vi "PathPlanner_Path_Equals.vi"(9 "Other Path":T1={"Reversed"=FALSE, "RotationTargets"=[], "ConstraintZones"=[], "EventMarkers"=[], "GlobalConstraints"={"MaxVelocityMps;"=0.0, "MaxAccelerationMpsSq;"=0.0, "MaxAngularVelRadPsEc;"=0.0, "MaxAngularAccRadPSecSq"=0.0, "Exists"=FALSE, "Unlimited"=FALSE, "NominalVoltageVolts"=12.0}, "GoalEndState"={"VelocityMPS"=0.0, "Rotation"={"VALUE"=0.0, "COS"=1.0, "SIN"=0.0}}, "AllPoints"=[], "Name"="", "Waypoints"=[], "PointTowardsZones"=[], "IdealStartingState"={"VelocityMPS"=0.0, "Rotation"={"VALUE"=1.0, "COS"=0.0, "SIN"=0.0}}, "IsChoreoPath"=FALSE, "PreventFlipping"=FALSE} {"IdealStartingState"."Rotation"."SIN" format="%13.4f"; "IdealStartingState"."Rotation"."COS" format="%13.4f"; "IdealStartingState"."Rotation"."VALUE" format="%13.4f"; "PointTowardsZones"."TargetPosition"."Y" format="%14.3f"; "PointTowardsZones"."TargetPosition"."X" format="%14.3f"; "PointTowardsZones"."RotationOffset"."SIN" format="%13.4f"; "PointTowardsZones"."RotationOffset"."COS" format="%13.4f"; "PointTowardsZones"."RotationOffset"."VALUE" format="%13.4f"; "Waypoints"."nextControl"."Y" format="%14.3f"; "Waypoints"."nextControl"."X" format="%14.3f"; "Waypoints"."anchor"."Y" format="%14.3f"; "Waypoints"."anchor"."X" format="%14.3f"; "Waypoints"."prevControl"."Y" format="%14.3f"; "Waypoints"."prevControl"."X" format="%14.3f"; "AllPoints"."RotationTarget"."rotation"."SIN" format="%13.4f"; "AllPoints"."RotationTarget"."rotation"."COS" format="%13.4f"; "AllPoints"."RotationTarget"."rotation"."VALUE" format="%13.4f"; "AllPoints"."Position"."Y" format="%14.3f"; "AllPoints"."Position"."X" format="%14.3f"; "GoalEndState"."Rotation"."SIN" format="%13.4f"; "GoalEndState"."Rotation"."COS" format="%13.4f"; "GoalEndState"."Rotation"."VALUE" format="%13.4f"; "RotationTargets"."rotation"."SIN" format="%13.4f"; "RotationTargets"."rotation"."COS" format="%13.4f"; "RotationTargets"."rotation"."VALUE" format="%13.4f"}, 11 "Path":T1={"Reversed"=FALSE, "RotationTargets"=[], "ConstraintZones"=[], "EventMarkers"=[], "GlobalConstraints"={"MaxVelocityMps;"=0.0, "MaxAccelerationMpsSq;"=0.0, "MaxAngularVelRadPsEc;"=0.0, "MaxAngularAccRadPSecSq"=0.0, "Exists"=FALSE, "Unlimited"=FALSE, "NominalVoltageVolts"=12.0}, "GoalEndState"={"VelocityMPS"=0.0, "Rotation"={"VALUE"=0.0, "COS"=1.0, "SIN"=0.0}}, "AllPoints"=[], "Name"="", "Waypoints"=[], "PointTowardsZones"=[], "IdealStartingState"={"VelocityMPS"=0.0, "Rotation"={"VALUE"=1.0, "COS"=0.0, "SIN"=0.0}}, "IsChoreoPath"=FALSE, "PreventFlipping"=FALSE} {"IdealStartingState"."Rotation"."SIN" format="%13.4f"; "IdealStartingState"."Rotation"."COS" format="%13.4f"; "IdealStartingState"."Rotation"."VALUE" format="%13.4f"; "PointTowardsZones"."TargetPosition"."Y" format="%14.3f"; "PointTowardsZones"."TargetPosition"."X" format="%14.3f"; "PointTowardsZones"."RotationOffset"."SIN" format="%13.4f"; "PointTowardsZones"."RotationOffset"."COS" format="%13.4f"; "PointTowardsZones"."RotationOffset"."VALUE" format="%13.4f"; "Waypoints"."nextControl"."Y" format="%14.3f"; "Waypoints"."nextControl"."X" format="%14.3f"; "Waypoints"."anchor"."Y" format="%14.3f"; "Waypoints"."anchor"."X" format="%14.3f"; "Waypoints"."prevControl"."Y" format="%14.3f"; "Waypoints"."prevControl"."X" format="%14.3f"; "AllPoints"."RotationTarget"."rotation"."SIN" format="%13.4f"; "AllPoints"."RotationTarget"."rotation"."COS" format="%13.4f"; "AllPoints"."RotationTarget"."rotation"."VALUE" format="%13.4f"; "AllPoints"."Position"."Y" format="%14.3f"; "AllPoints"."Position"."X" format="%14.3f"; "GoalEndState"."Rotation"."SIN" format="%13.4f"; "GoalEndState"."Rotation"."COS" format="%13.4f"; "GoalEndState"."Rotation"."VALUE" format="%13.4f"; "RotationTargets"."rotation"."SIN" format="%13.4f"; "RotationTargets"."rotation"."COS" format="%13.4f"; "RotationTargets"."rotation"."VALUE" format="%13.4f"}) -> (3 "Equals":bool)   [LabVIEW 2019, in "PathPlanner24.lvlib"]
doc: "Determines if two paths are identical.\n\nNote: Reversed and PreviewEndState are not part of the comparison\n\nInputs:\n - Path Path - Data structure containing path definition\n - OtherPath - Path - Data structure containing path definition\n\nOutputs:\n - Equal - boolean - TRUE if paths are identical."
uses:
  PathPlanner24.lvlib
  <vilib>/Rock Robotics/WPI/ThirdParty/JAS_Junk/TrajLib/TypeDef/TRANSLATION2D.ctl
  <vilib>/Rock Robotics/WPI/ThirdParty/JAS_Junk/TrajLib/Trajectory_Library.lvlib
  <vilib>/Rock Robotics/WPI/ThirdParty/JAS_Junk/TrajLib/TypeDef/ROTATION2D.ctl
  TypeDef/PathPlannerRotationTarget.ctl
  TypeDef/PathPlannerPathConstraints.ctl
  TypeDef/PathPlannerConstraintsZone.ctl
  TypeDef/PathPlannerCommandUtil.ctl
  TypeDef/PathPlannerEventMarker.ctl
  TypeDef/PathPlannerGoalEndState.ctl
  TypeDef/PathPlannerPathPoint.ctl
  TypeDef/PathPlannerPath.ctl
  ENum/PathPlanner_TrajectoryEvent_Type_ENUM.ctl
  TypeDef/PathPlannerWaypoint.ctl
  TypeDef/PathPlannerPointTowardsZone.ctl
  TypeDef/PathPlannerIdealStartingState.ctl
  ENum/PathPlanner_CommandUtil_Type_ENUM.ctl
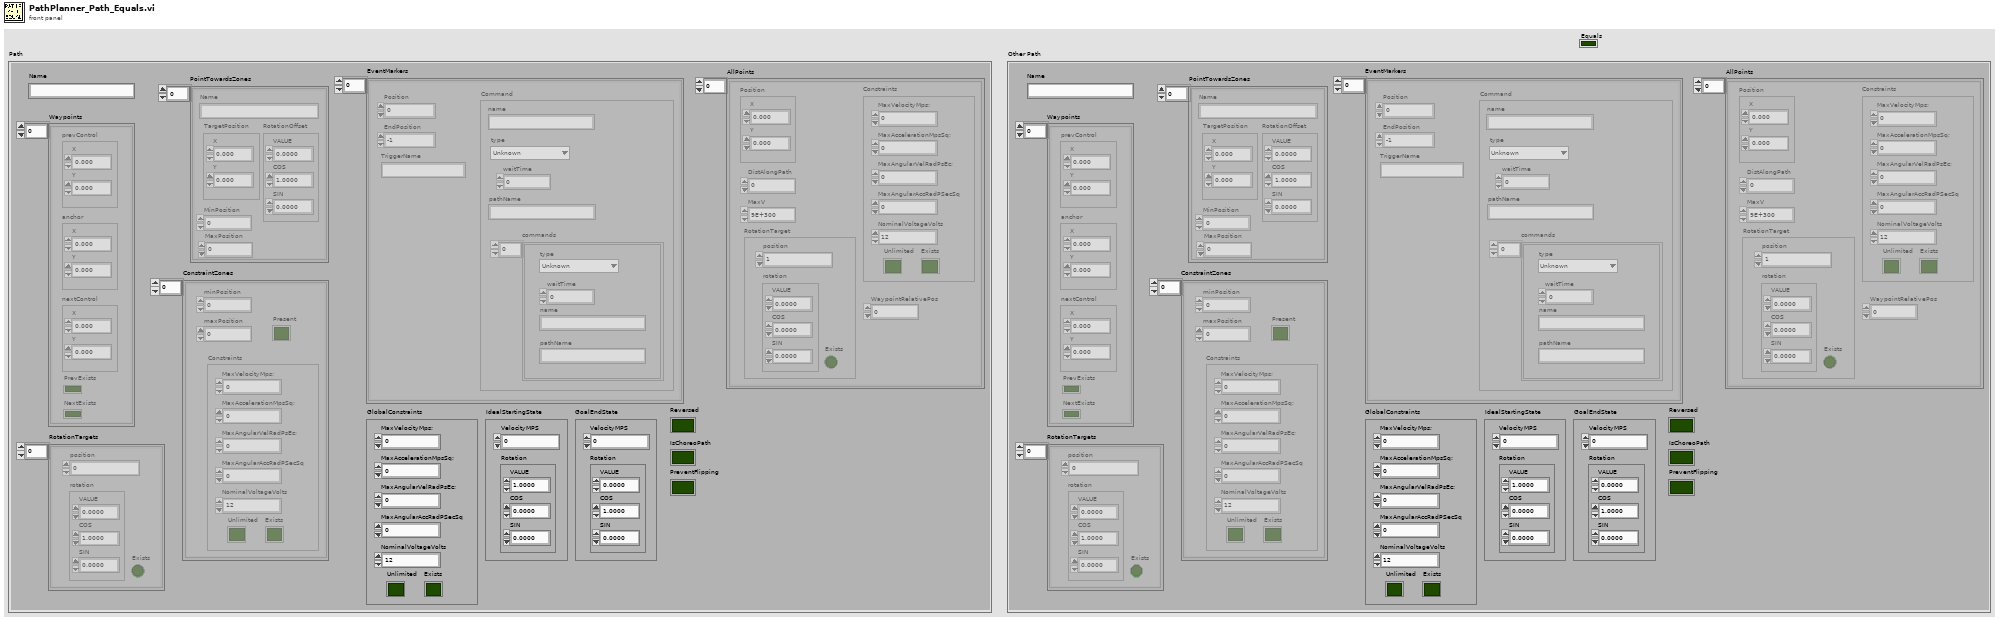
[diagram p1: front panel]
types:
  T1 = typedef "PathPlanner24.lvlib/PathPlannerPath.ctl" = cluster{"Reversed":bool, "RotationTargets":T2[], "ConstraintZones":T4[], "EventMarkers":T6[], "GlobalConstraints":T5, "GoalEndState":T10, "AllPoints":T11[], "Name":string, "Waypoints":T13[], "PointTowardsZones":T14[], "IdealStartingState":T15, "IsChoreoPath":bool, "PreventFlipping":bool}
  T2 = typedef "PathPlanner24.lvlib/PathPlannerRotationTarget.ctl" = cluster{"position":dbl, "rotation":T3, "Exists":bool}
  T3 = typedef "Trajectory_Library.lvlib/ROTATION2D.ctl" = cluster{"VALUE":dbl, "COS":dbl, "SIN":dbl}
  T4 = typedef "PathPlanner24.lvlib/PathPlannerConstraintsZone.ctl" = cluster{"minPosition":dbl, "maxPosition":dbl, "Constraints":T5, "Present":bool}
  T5 = typedef "PathPlanner24.lvlib/PathPlannerPathConstraints.ctl" = cluster{"MaxVelocityMps;":dbl, "MaxAccelerationMpsSq;":dbl, "MaxAngularVelRadPsEc;":dbl, "MaxAngularAccRadPSecSq":dbl, "Exists":bool, "Unlimited":bool, "NominalVoltageVolts":dbl}
  T6 = typedef "PathPlanner24.lvlib/PathPlannerEventMarker.ctl" = cluster{"Position":dbl, "Command":T7, "TriggerName":string, "EndPosition":dbl}
  T7 = typedef "PathPlanner24.lvlib/PathPlannerCommandUtil.ctl" = cluster{"waitTime":dbl, "name":string, "pathName":string, "commands":cluster{"type":T8, "waitTime":dbl, "name":string, "pathName":string}[], "type":T9}
  T8 = typedef "PathPlanner24.lvlib/PathPlanner_TrajectoryEvent_Type_ENUM.ctl" = enum16{"Unknown", "Wait", "Named", "Path", "Sequential", "Parallel", "Race", "Deadline", "PointTowardsZoneEnter", "PointTowardsZoneExit", "TriggerEventStart", "TriggerEventStop", "TriggerEventOneshot"}
  T9 = typedef "PathPlanner24.lvlib/PathPlanner_CommandUtil_Type_ENUM.ctl" = enum16{"Unknown", "Wait", "Named", "Path", "Sequential", "Parallel", "Race", "Deadline"}
  T10 = typedef "PathPlanner24.lvlib/PathPlannerGoalEndState.ctl" = cluster{"VelocityMPS":dbl, "Rotation":T3}
  T11 = typedef "PathPlanner24.lvlib/PathPlannerPathPoint.ctl" = cluster{"Position":T12, "DistAlongPath":dbl, "MaxV":dbl, "Constraints":T5, "RotationTarget":T2, "WaypointRelativePos":dbl}
  T12 = typedef "Trajectory_Library.lvlib/TRANSLATION2D.ctl" = cluster{"X":dbl, "Y":dbl}
  T13 = typedef "PathPlanner24.lvlib/PathPlannerWaypoint.ctl" = cluster{"prevControl":T12, "anchor":T12, "nextControl":T12, "PrevExists":bool, "NextExists":bool}
  T14 = typedef "PathPlanner24.lvlib/PathPlannerPointTowardsZone.ctl" = cluster{"RotationOffset":T3, "Name":string, "TargetPosition":T12, "MinPosition":dbl, "MaxPosition":dbl}
  T15 = typedef "PathPlanner24.lvlib/PathPlannerIdealStartingState.ctl" = cluster{"VelocityMPS":dbl, "Rotation":T3}
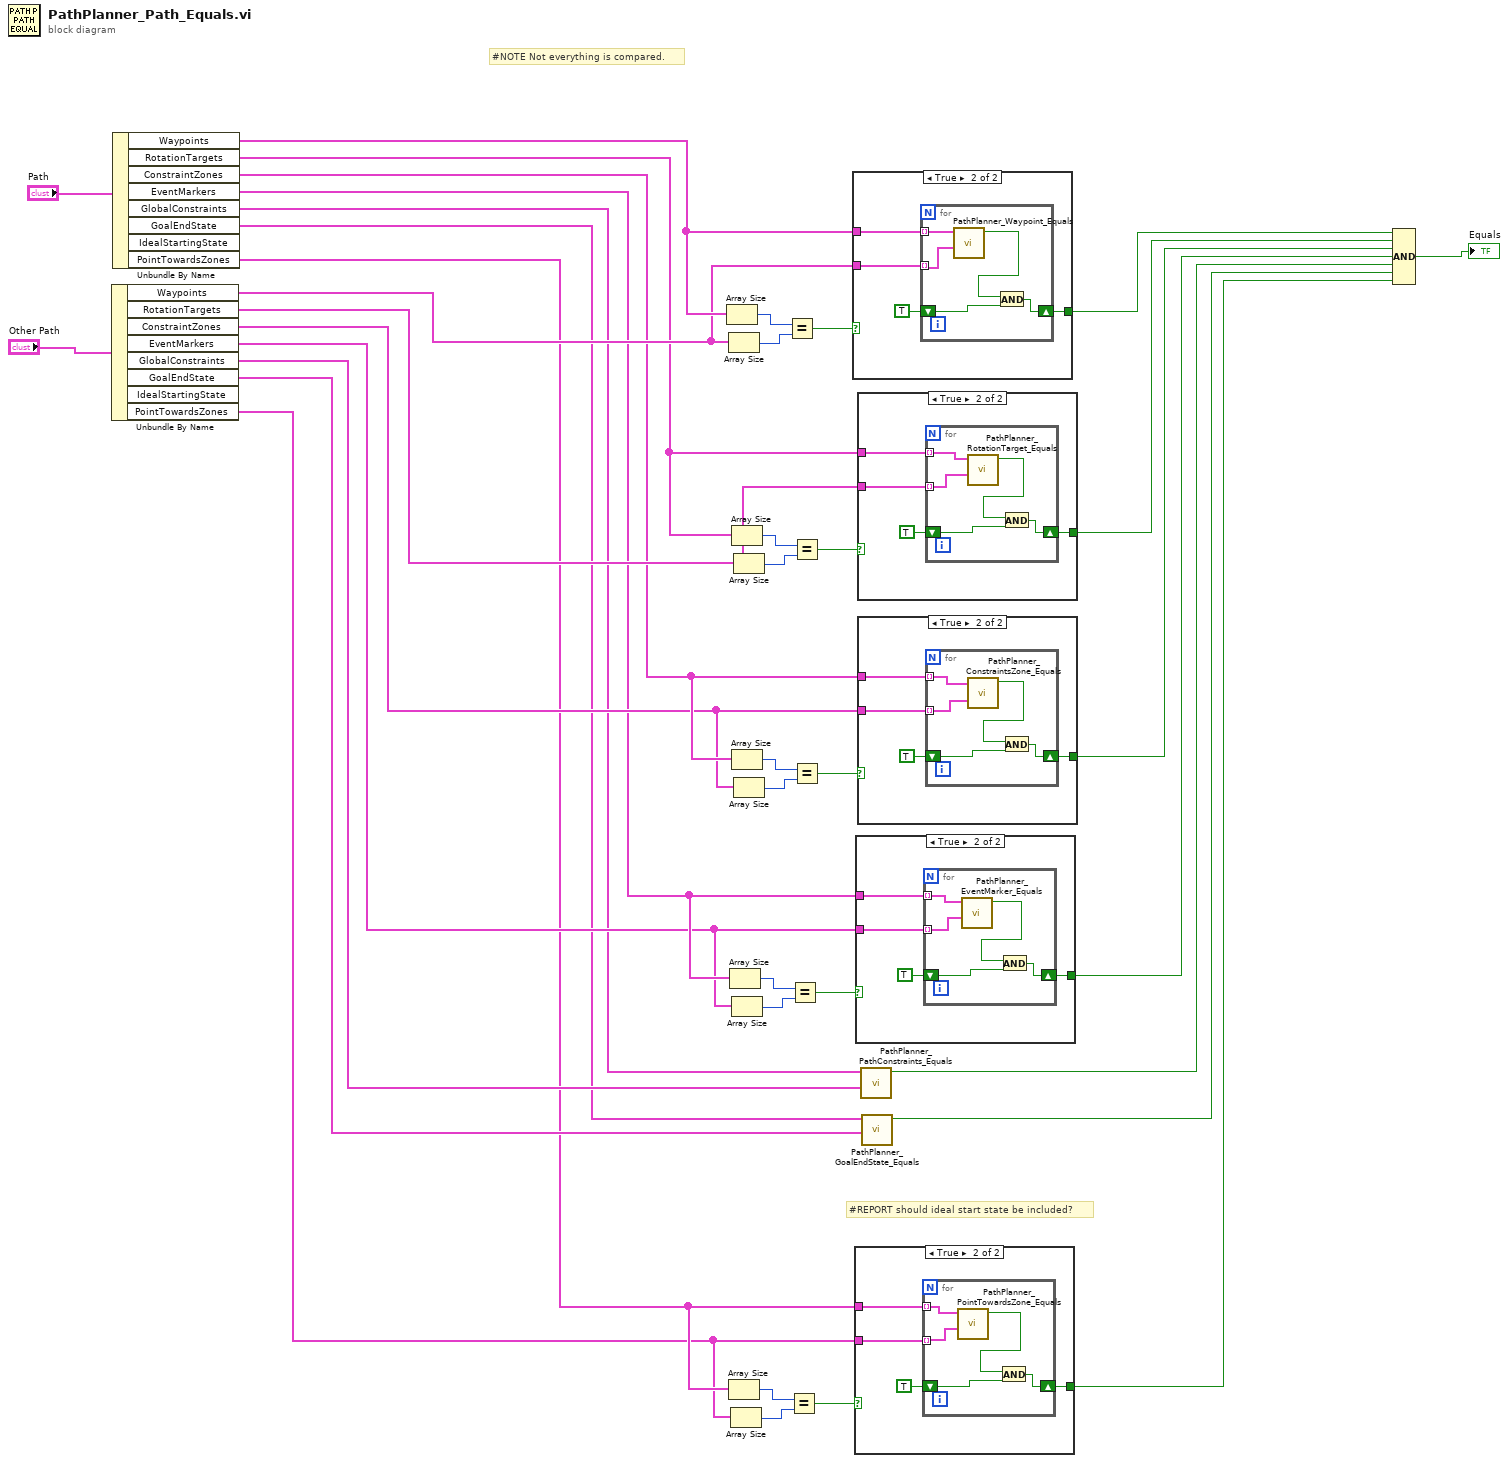
[diagram p0: block diagram]
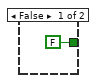
[diagram p2: hidden frame]
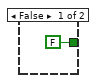
[diagram p3: hidden frame]
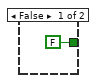
[diagram p4: hidden frame]
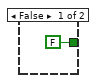
[diagram p5: hidden frame]
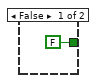
[diagram p6: hidden frame]
diagram:
  # "#REPORT should ideal start state be included?"
  # "#NOTE Not everything is compared."
  n1 = Unbundle By Name("Other Path") -> ("Waypoints"=w33:T13[], "RotationTargets"=w26:T2[], "ConstraintZones"=w20:T4[], "EventMarkers"=w14:T6[], "GlobalConstraints"=w11:T5, "GoalEndState"=w8:T10, "PointTowardsZones"=w2:T14[])  [unwired: 1 out]
  n2 = Unbundle By Name("Path") -> ("Waypoints"=w34:T13[], "RotationTargets"=w27:T2[], "ConstraintZones"=w21:T4[], "EventMarkers"=w15:T6[], "GlobalConstraints"=w12:T5, "GoalEndState"=w9:T10, "PointTowardsZones"=w3:T14[])  [unwired: 1 out]
  n3 = Array Size(array=w34) -> (size(s)=w37:i32)
  n4 = Array Size(array=w33) -> (size(s)=w36:i32)
  n5 = Array Size(array=w3) -> (size(s)=w6:i32)
  n6 = Array Size(array=w15) -> (size(s)=w18:i32)
  n7 = Array Size(array=w2) -> (size(s)=w5:i32)
  n8 = Array Size(array=w27) -> (size(s)=w30:i32)
  n9 = Array Size(array=w21) -> (size(s)=w24:i32)
  n10 = Array Size(array=w14) -> (size(s)=w17:i32)
  n11 = Array Size(array=w26) -> (size(s)=w29:i32)
  n12 = Array Size(array=w20) -> (size(s)=w23:i32)
  n13 = Equal?(x=w37, y=w36) -> (x = y?=w35:bool)
  n14 = Equal?(x=w6, y=w5) -> (x = y?=w4:bool)
  n15 = Equal?(x=w18, y=w17) -> (x = y?=w16:bool)
  n16 = Equal?(x=w30, y=w29) -> (x = y?=w28:bool)
  n17 = Equal?(x=w24, y=w23) -> (x = y?=w22:bool)
  n18 = case shown="True" w35 {
    tunnel: w34 -> [_ w43]
    tunnel: w33 -> [_ w42]
    tunnel: [FALSE w41] -> w32
    frame False {
    }
    frame True {
      n19 = for {
        shift-right: [w49] -> w41
        shift-left: TRUE -> [w48]
        tunnel: w43 -> [w47] mode=indexing
        tunnel: w42 -> [w46] mode=indexing
        n20 = call "PathPlanner_Waypoint_Equals.vi"("Other Waypoint"=w46, "PathPlannerWaypoint"=w47) -> ("Equal"=w45:bool)  [unwired: 9 in]
        n21 = And(x=w45, y=w48) -> (x .and. y?=w49:bool)
      }
    }
  }
  n22 = case shown="True" w4 {
    tunnel: w3 -> [_ w53]
    tunnel: w2 -> [_ w52]
    tunnel: [FALSE w51] -> w1
    frame False {
    }
    frame True {
      n23 = for {
        shift-right: [w59] -> w51
        shift-left: TRUE -> [w58]
        tunnel: w53 -> [w57] mode=indexing
        tunnel: w52 -> [w56] mode=indexing
        n24 = call "PathPlanner_PointTowardsZone_Equals.vi"("OtherPointTowardsZone"=w56, "PointTowardsZone"=w57) -> ("Equals"=w55:bool)  [unwired: 9 in]
        n25 = And(x=w55, y=w58) -> (x .and. y?=w59:bool)
      }
    }
  }
  n26 = case shown="True" w16 {
    tunnel: w15 -> [_ w63]
    tunnel: w14 -> [_ w62]
    tunnel: [FALSE w61] -> w13
    frame False {
    }
    frame True {
      n27 = for {
        shift-right: [w69] -> w61
        shift-left: TRUE -> [w68]
        tunnel: w63 -> [w67] mode=indexing
        tunnel: w62 -> [w66] mode=indexing
        n28 = call "PathPlanner_EventMarker_Equals.vi"("Other EventMarker"=w66, "EventMarker"=w67) -> ("Equal"=w65:bool)  [unwired: 9 in]
        n29 = And(x=w65, y=w68) -> (x .and. y?=w69:bool)
      }
    }
  }
  n30 = case shown="True" w28 {
    tunnel: w27 -> [_ w73]
    tunnel: w26 -> [_ w72]
    tunnel: [FALSE w71] -> w25
    frame False {
    }
    frame True {
      n31 = for {
        shift-right: [w79] -> w71
        shift-left: TRUE -> [w78]
        tunnel: w73 -> [w77] mode=indexing
        tunnel: w72 -> [w76] mode=indexing
        n32 = call "PathPlanner_RotationTarget_Equals.vi"("Other GoalEndState"=w76, "RotationTarget"=w77) -> ("Equal"=w75:bool)  [unwired: 9 in]
        n33 = And(x=w75, y=w78) -> (x .and. y?=w79:bool)
      }
    }
  }
  n34 = case shown="True" w22 {
    tunnel: w21 -> [_ w83]
    tunnel: w20 -> [_ w82]
    tunnel: [FALSE w81] -> w19
    frame False {
    }
    frame True {
      n35 = for {
        shift-right: [w89] -> w81
        shift-left: TRUE -> [w88]
        tunnel: w83 -> [w87] mode=indexing
        tunnel: w82 -> [w86] mode=indexing
        n36 = call "PathPlanner_ConstraintsZone_Equals.vi"("Other Constraints Zone"=w86, "ConstraintsZone"=w87) -> ("Equal"=w85:bool)  [unwired: 9 in]
        n37 = And(x=w85, y=w88) -> (x .and. y?=w89:bool)
      }
    }
  }
  n38 = call "PathPlanner_PathConstraints_Equals.vi"("Other PathPlannerConstraints"=w11, "PathPlannerConstraints"=w12) -> ("Equal"=w10:bool)  [unwired: 9 in]
  n39 = call "PathPlanner_GoalEndState_Equals.vi"("Other GoalEndState"=w8, "GoalEndState"=w9) -> ("Equal"=w7:bool)  [unwired: 9 in]
  n40 = Compound Arithmetic op=AND(w32, w25, w19, w13, w10, w7, w1) -> (→"Equals":bool)
